vi "XNET CAN Write.vi"() -> ()   [LabVIEW 2021]
uses:
  <vilib>/CIF Foundation/CIF CAN RW Core/typedef/CAN Port Configuration.ctl
  <vilib>/CIF Foundation/CIF CAN RW Core/typedef/CAN Mode.ctl
  <vilib>/CIF Foundation/CIF CAN RW Core/typedef/FD Config.ctl
  <vilib>/xnet/xnet.llb/XNET Frame CAN.ctl
  <vilib>/xnet/xnet.llb/XNET Frame Type CAN.ctl
  <vilib>/CIF Foundation/CIF XNET CAN RW/XNET CAN RW.lvclass
  C:/Program Files/National Instruments/LabVIEW 2021/vi.lib/CIF Foundation/CIF CAN RW Core/CAN_RW_CORE.lvclass
  <vilib>/CIF Foundation/CIF CAN RW Core/CAN_RW_CORE.lvclass/CAN_RW_CORE.ctl
  <vilib>/CIF Foundation/CIF PCAP Parse and Build/pcap_Parse_Build_CIF.lvclass/pcap_Parse_Build_CIF.ctl
  <vilib>/CIF Foundation/CIF Utilities/Time/System Time/LabVIEW Time to TAI Time.vi
  <vilib>/CIF Foundation/CIF XNET CAN RW/Utilities/XNET CAN to Header Cluster.vi
  <vilib>/CIF Foundation/CIF PCAP Parse and Build/Build/Build Packet Header.vi
  <vilib>/CIF Foundation/CIF PCAP Parse and Build/Build/SubVIs/Flatten SocketCAN Header.vi
  <vilib>/CIF Foundation/CIF CAN RW Core/Utilities/Filter Packets.vi
  <vilib>/CIF Foundation/CIF CAN RW Core/Accessors/Read CAN Interface Mode.vi
  <vilib>/CIF Foundation/CIF CAN RW Core/Accessors/Read pcap class.vi
  <vilib>/CIF Foundation/CIF PCAP Parse and Build/Build/SubVIs/Flatten Packet Header.vi
  <vilib>/CIF Foundation/CIF Utilities/DataTypes/Flatten Unflatten/Flatten U32.vi
  <vilib>/CIF Foundation/CIF PCAP Parse and Build/pcap_Parse_Build_CIF.lvclass
  <vilib>/CIF Foundation/CIF Utilities/Time/Time_CIF_U.lvlib
  <vilib>/CIF Foundation/CIF Utilities/DataTypes/DataTypes_CIF_U.lvlib
  <vilib>/CIF Foundation/CIF CAN RW Core/CAN_RW_CORE.lvclass
panel:
  in  "Use Benchmark Payload":bool
  in  "Loop rate (ms)":u32=100
  in  "stop":bool
  in  "XNET CAN Data":T1[](array[typedef])=[{"timestamp"=timestamp(3831573600 s since 1904-01-01), "payload"=[1, 2, 3, 4, 5, 6, 7, 8], "identifier"=33, "type"=16, "extended?"=TRUE, "echo?"=FALSE}, {"timestamp"=timestamp(3831570000 s since 1904-01-01), "payload"=[10, 11, 10, 13, 11, 10, 11, 14], "identifier"=82, "type"=0, "extended?"=TRUE, "echo?"=FALSE}] {"payload" format="%x"; "timestamp" format="%<%.7X\n%x>T"; "type" items=["CAN Data"=0, "CAN Remote"=1, "CAN Bus Error"=2, "CAN 2.0 Data"=8, "CAN FD Data"=16, "CAN FD+BRS Data"=24, "J1939 Data"=192, "Delay"=224, "Log Trigger"=225, "Start Trigger"=226]; "identifier" format="%x"}
  out "error out":errorcluster
  in  "Port Configuration":T3={"Mode"=enum."CAN FD", "Baud Rate"=500000, "Temination On"=TRUE, "Subordinate"=FALSE, "Echo TX"=FALSE, "FD Config"={"FD Baud Rate"=2000000, "ISO Mode"=TRUE, "BRS Enabled"=TRUE}} {"FD Config"."FD Baud Rate" format="%.0p"; "Baud Rate" format="%.0p"}
  in  "TX Interface":string="CAN1"
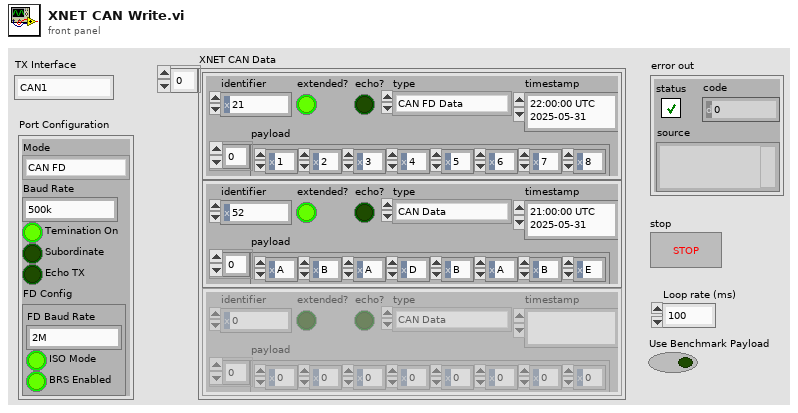
[diagram p1: front panel]
types:
  T1 = typedef "XNET Frame CAN.ctl" = cluster{"timestamp":timestamp, "payload":u8[], "identifier":u32, "type":T2, "extended?":bool, "echo?":bool}
  T2 = typedef "XNET Frame Type CAN.ctl" = u8
  T3 = typedef "CAN_RW_CORE.lvclass/CAN Port Configuration.ctl" = cluster{"Mode":T4, "Baud Rate":u64, "Temination On":bool, "Subordinate":bool, "Echo TX":bool, "FD Config":T5}
  T4 = typedef "CAN_RW_CORE.lvclass/CAN Mode.ctl" = enum16{"CAN 2.0", "CAN FD"}
  T5 = typedef "CAN_RW_CORE.lvclass/FD Config.ctl" = cluster{"FD Baud Rate":u64, "ISO Mode":bool, "BRS Enabled":bool}
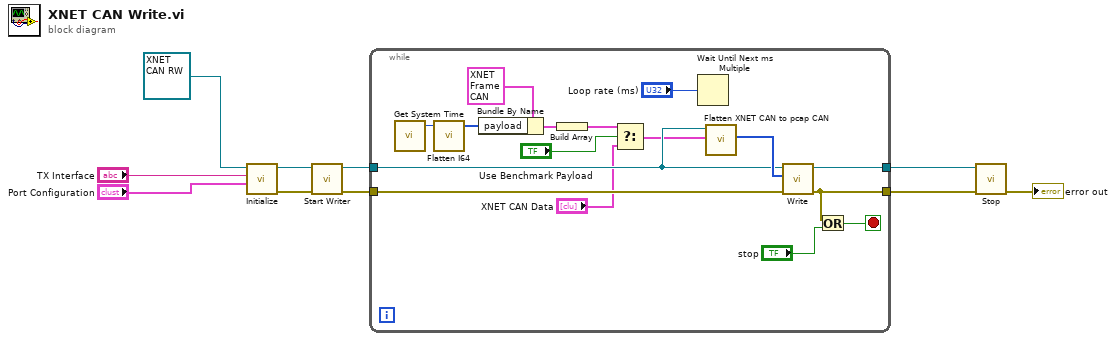
[diagram p0: block diagram]
diagram:
  n1 = call <vilib>:"Initialize.vi"("Port Configuration"="Port Configuration", "Interface"="TX Interface", "XNET_CAN_RW in"=refnum<class "XNET CAN RW.lvclass"> refnum ("CAN_Logic in")) -> ("error out"=w2:errorcluster, "XNET_CAN_RW out"=w4:refnum<class "XNET CAN RW.lvclass">)  [unwired: 7 in]
  n2 = call-dynamic "Start Writer.vi"("error in (no error)"=w2, "XNET_CAN_RW in"=w4) -> ("error out"=w10:errorcluster, "XNET_CAN_RW out"=w3:refnum<class "XNET CAN RW.lvclass">)  [unwired: 8 in]
  n3 = while {
    tunnel: w10 -> [w26]
    tunnel: [w21] -> w1
    tunnel: w3 -> [w23]
    tunnel: [w25] -> w9
    stop <- w19 stop-if-true
    n4 = call <vilib>:"Get System Time.vi"() -> ("Time (ns)"=w16:i64)  [unwired: 5 in]
    n5 = call <vilib>:"Flatten I64.vi"("I64"=w16) -> ("Flat Data"=w15:u8[])  [unwired: 4 in]
    n6 = Bundle By Name(cluster=T1 {"timestamp"=timestamp(3831573600 s since 1904-01-01), "payload"=[1, 2, 3, 4, 5, 6, 7, 8], "identifier"=33, "type"=16, "extended?"=TRUE, "echo?"=FALSE} ("CAN frame"), "payload"=w15) -> (w18:T1)
    n7 = Build Array(w18) -> (w13:T1[])
    n8 = Select(t=w13, s="Use Benchmark Payload", f="XNET CAN Data") -> (s? t:f=w14:T1[])
    n9 = Wait Until Next ms Multiple(millisecond multiple="Loop rate (ms)") -> ()  [unwired: 1 out]
    n10 = call <vilib>:"Flatten XNET CAN to pcap CAN.vi"("XNET CAN Data"=w14, "XNET_CAN_RW in"=w23) -> ("pcap CAN DATA"=w24:u8[])  [unwired: 7 in, 2 out]
    n11 = call-dynamic "Write.vi"("error in (no error)"=w26, "pcap CAN DATA in"=w24, "XNET_CAN_RW in"=w23) -> ("error out"=w21:errorcluster, "XNET_CAN_RW out"=w25:refnum<class "XNET CAN RW.lvclass">)  [unwired: 6 in, 1 out]
    n12 = Or(x=w21, y="stop") -> (x .or. y?=w19:bool)
  }
  n13 = call-dynamic "Stop.vi"("error in (no error)"=w1, "XNET_CAN_RW in"=w9) -> ("error out"=→"error out":errorcluster)  [unwired: 8 in, 1 out]
